vi "RT Main.vi"() -> ()   [LabVIEW 2025]
doc: "This template is for the Queued Message Handler design pattern.\n\nThe Event Handling Loop generates messages based on user interface actions.\n\nThe Message Handling Loop processes messages generated by the Event Handling Loop, or by other messages. The messages are string values, so new messages can be added easily to the Message Cases case structure in the Message Handling Loop. Each message cluster can also provide an optional value for Message Data, which is a variant that can be converted to whatever message-specific data is required."
uses:
  support/Message Queue/Message Queue.lvlib
  controls/Raw Values.ctl
  controls/Control Configuration.ctl
  controls/Control State.ctl
  Globals/Global - Configuration Options.vi
  Globals/Global - RT Stream Connections.vi
  controls/Functional Global Operation.ctl
  C:/40T/controls/Control State.ctl
  <vilib>/nisyscfg/nisyscfg.lvlib
  C:/40T/controls/ProfiBusData.ctl
  controls/ProfiBusData.ctl
panel:
  out "cluster":T1
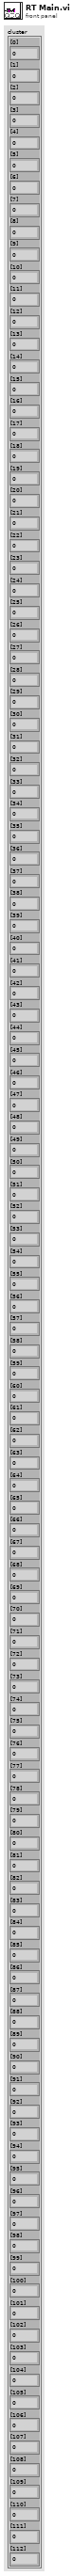
[diagram p1: front panel]
types:
  T1 = typedef "ProfiBusData.ctl" = cluster{"[0]":dbl, "[1]":dbl, "[2]":dbl, "[3]":dbl, "[4]":dbl, "[5]":dbl, "[6]":dbl, "[7]":dbl, "[8]":dbl, "[9]":dbl, "[10]":dbl, "[11]":dbl, "[12]":dbl, "[13]":dbl, "[14]":dbl, "[15]":dbl, "[16]":dbl, "[17]":dbl, "[18]":dbl, "[19]":dbl, "[20]":dbl, "[21]":dbl, "[22]":dbl, "[23]":dbl, "[24]":dbl, "[25]":dbl, "[26]":dbl, "[27]":dbl, "[28]":dbl, "[29]":dbl, "[30]":dbl, "[31]":dbl, "[32]":dbl, "[33]":dbl, "[34]":dbl, "[35]":dbl, "[36]":dbl, "[37]":dbl, "[38]":dbl, "[39]":dbl, "[40]":dbl, "[41]":dbl, "[42]":dbl, "[43]":dbl, "[44]":dbl, "[45]":dbl, "[46]":dbl, "[47]":dbl, "[48]":dbl, "[49]":dbl, "[50]":dbl, "[51]":dbl, "[52]":dbl, "[53]":dbl, "[54]":dbl, "[55]":dbl, "[56]":dbl, "[57]":dbl, "[58]":dbl, "[59]":dbl, "[60]":dbl, "[61]":dbl, "[62]":dbl, "[63]":dbl, "[64]":dbl, "[65]":dbl, "[66]":dbl, "[67]":dbl, "[68]":dbl, "[69]":dbl, "[70]":dbl, "[71]":dbl, "[72]":dbl, "[73]":dbl, "[74]":dbl, "[75]":dbl, "[76]":dbl, "[77]":dbl, "[78]":dbl, "[79]":dbl, "[80]":dbl, "[81]":dbl, "[82]":dbl, "[83]":dbl, "[84]":dbl, "[85]":dbl, "[86]":dbl, "[87]":dbl, "[88]":dbl, "[89]":dbl, "[90]":dbl, "[91]":dbl, "[92]":dbl, "[93]":dbl, "[94]":dbl, "[95]":dbl, "[96]":dbl, "[97]":dbl, "[98]":dbl, "[99]":dbl, "[100]":dbl, "[101]":dbl, "[102]":dbl, "[103]":dbl, "[104]":dbl, "[105]":dbl, "[106]":dbl, "[107]":dbl, "[108]":dbl, "[109]":dbl, "[110]":dbl, "[111]":dbl, "[112]":dbl}
  T2 = typedef "Functional Global Operation.ctl" = enum16{"Initialize", "Read", "Write"}
  T3 = typedef "Control State.ctl" = enum16{"Safe State", "Control (PID)"}
  T4 = typedef "Raw Values.ctl" = cluster{"Channel 0":dbl, "Channel 1":dbl, "Channel 2":dbl, "Channel 3":dbl}
  T5 = typedef "Control Configuration.ctl" = cluster{"PID Gains":cluster{"proportional gain (Kc)":dbl, "integral gain (Kc*Ts/Ti)":dbl, "derivative gain (Kc*Td/Ts)":dbl}, "Output Range":cluster{"output high":dbl, "output low":dbl}}
  T6 = typedef "All Control Configuration Values.ctl" = cluster{"Control State":T3, "Setpoints":T4, "Control Configurations":T5[], "Temperature Thresholds":dbl[]}
  T7 = cluster{"[0]":dbl, "[1]":dbl, "[2]":dbl, "[3]":dbl, "[4]":dbl, "[5]":dbl, "[6]":dbl, "[7]":dbl, "[8]":dbl, "[9]":dbl, "[10]":dbl, "[11]":dbl, "[12]":dbl, "[13]":dbl, "[14]":dbl, "[15]":dbl, "[16]":dbl, "[17]":dbl, "[18]":dbl, "[19]":dbl, "[20]":dbl, "[21]":dbl, "[22]":dbl, "[23]":dbl, "[24]":dbl, "[25]":dbl, "[26]":dbl, "[27]":dbl, "[28]":dbl, "[29]":dbl, "[30]":dbl, "[31]":dbl, "[32]":dbl, "[33]":dbl, "[34]":dbl, "[35]":dbl, "[36]":dbl, "[37]":dbl, "[38]":dbl, "[39]":dbl, "[40]":dbl, "[41]":dbl, "[42]":dbl, "[43]":dbl, "[44]":dbl, "[45]":dbl, "[46]":dbl, "[47]":dbl, "[48]":dbl, "[49]":dbl, "[50]":dbl, "[51]":dbl, "[52]":dbl, "[53]":dbl, "[54]":dbl, "[55]":dbl, "[56]":dbl, "[57]":dbl, "[58]":dbl, "[59]":dbl, "[60]":dbl, "[61]":dbl, "[62]":dbl, "[63]":dbl, "[64]":dbl, "[65]":dbl, "[66]":dbl, "[67]":dbl, "[68]":dbl, "[69]":dbl, "[70]":dbl, "[71]":dbl, "[72]":dbl, "[73]":dbl, "[74]":dbl, "[75]":dbl, "[76]":dbl, "[77]":dbl, "[78]":dbl, "[79]":dbl, "[80]":dbl, "[81]":dbl, "[82]":dbl, "[83]":dbl, "[84]":dbl, "[85]":dbl, "[86]":dbl, "[87]":dbl, "[88]":dbl, "[89]":dbl, "[90]":dbl, "[91]":dbl, "[92]":dbl, "[93]":dbl, "[94]":dbl, "[95]":dbl, "[96]":dbl, "[97]":dbl, "[98]":dbl, "[99]":dbl, "[100]":dbl, "[101]":dbl, "[102]":dbl, "[103]":dbl, "[104]":dbl, "[105]":dbl, "[106]":dbl, "[107]":dbl, "[108]":dbl, "[109]":dbl, "[110]":dbl, "[111]":dbl, "[112]":dbl}
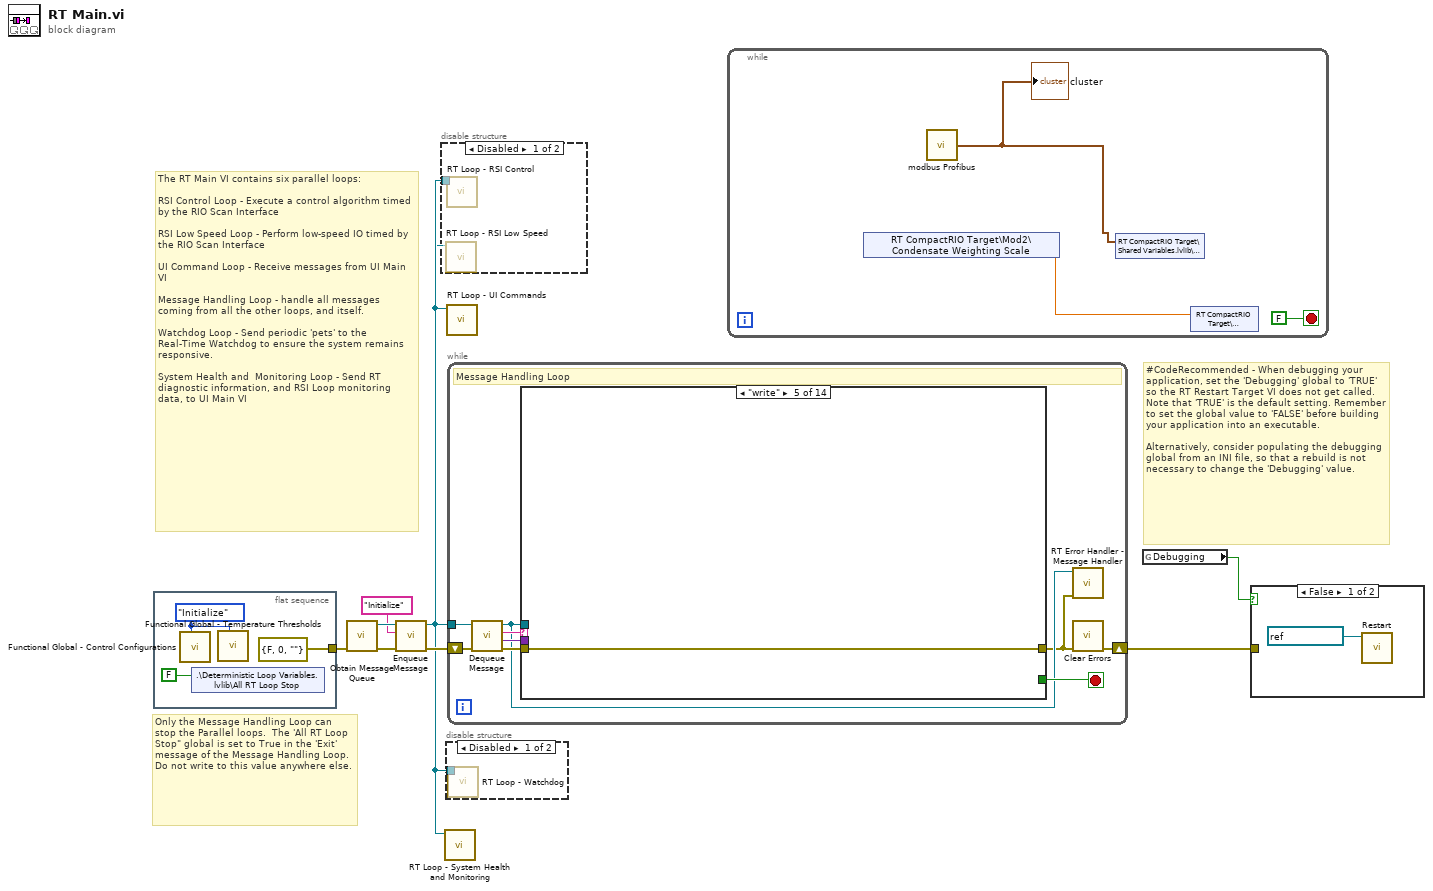
[diagram p0: block diagram]
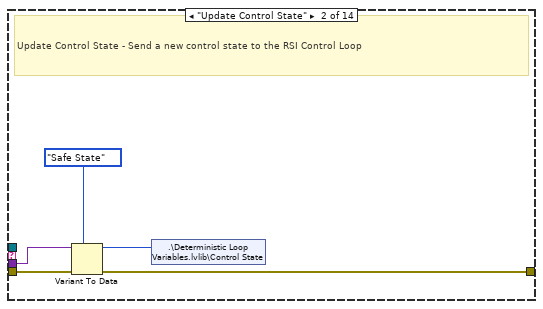
[diagram p6: hidden frame]
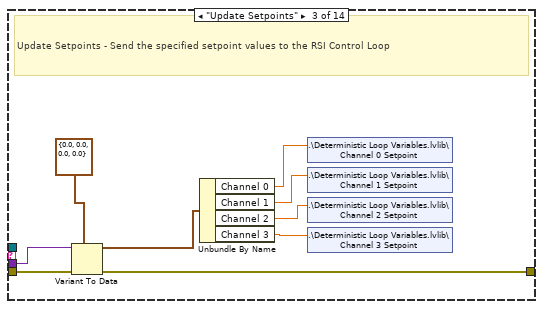
[diagram p7: hidden frame]
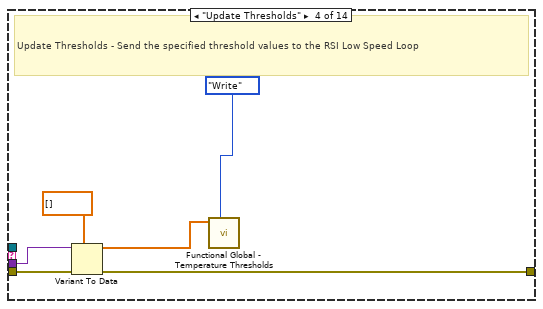
[diagram p8: hidden frame]
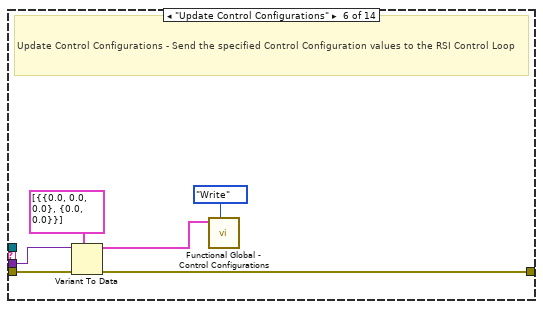
[diagram p9: hidden frame]
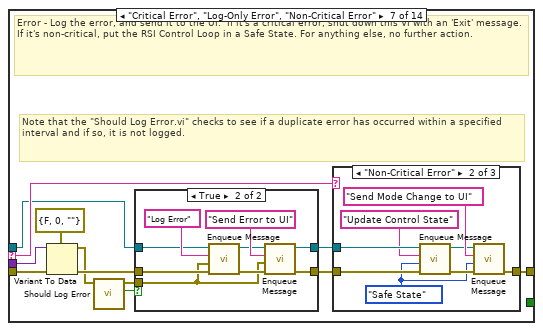
[diagram p10: hidden frame]
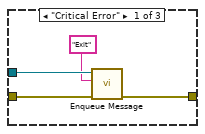
[diagram p12: hidden frame]
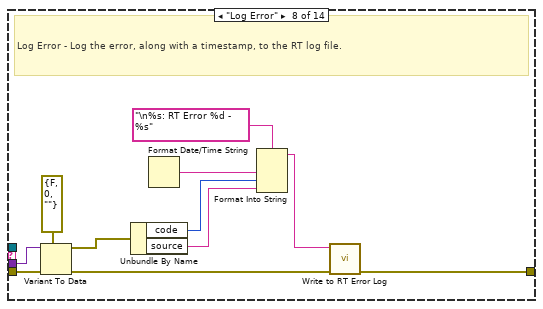
[diagram p14: hidden frame]
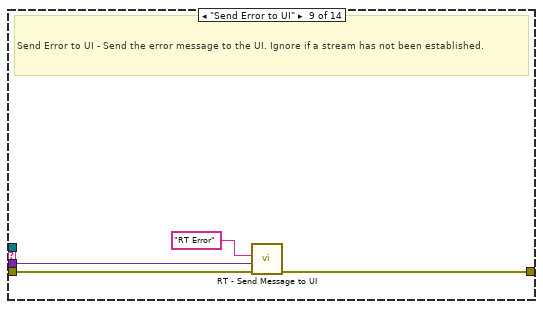
[diagram p15: hidden frame]
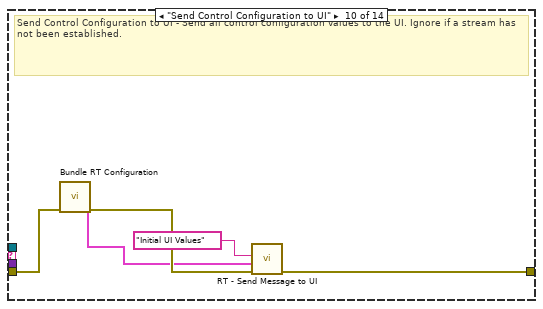
[diagram p16: hidden frame]
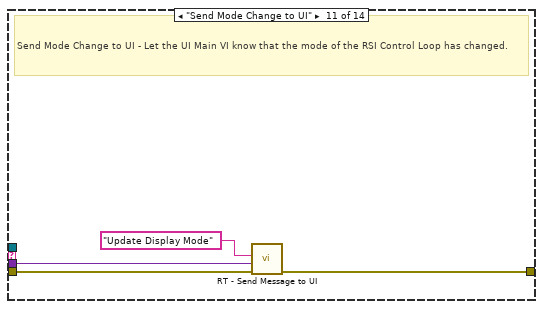
[diagram p17: hidden frame]
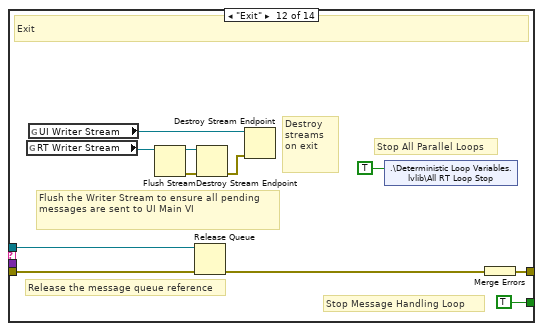
[diagram p18: hidden frame]
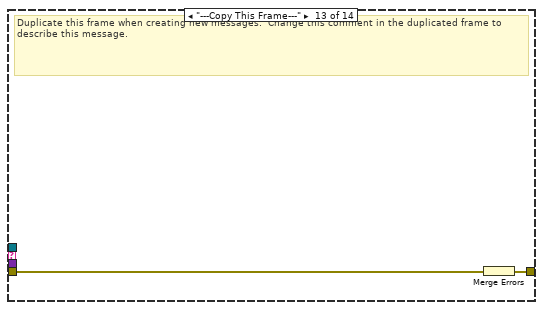
[diagram p19: hidden frame]
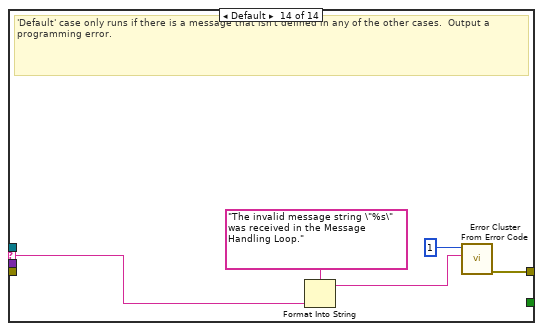
[diagram p20: hidden frame]
diagram:
  # "#CodeRecommended - When debugging your application, set the 'Debugging' global to 'TRUE' so the RT Restart Target VI does not get called.  Note that 'TRUE' is the default setting. Remember to set the global value to 'FALSE' before building your application into an executable.\n\nAlternatively, consider populating the debugging global from an INI file, so that a rebuild is not necessary to change the 'Debugging' value."
  # "The RT Main VI contains six parallel loops:\n\nRSI Control Loop - Execute a control algorithm timed by the RIO Scan Interface\n\nRSI Low Speed Loop - Perform low-speed IO timed by the RIO Scan Interface\n\nUI Command Loop - Receive messages from UI Main VI\n\nMessage Handling Loop - handle all messages coming from all the other loops, and itself.\n\nWatchdog Loop - Send periodic 'pets' to the Real-Time Watchdog to ensure the system remains responsive.\n\nSystem Health and  Monitoring Loop - Send RT diagnostic information, and RSI Loop monitoring data, to UI Main VI"
  # "Only the Message Handling Loop can stop the Parallel loops.  The 'All RT Loop Stop\" global is set to True in the 'Exit' message of the Message Handling Loop.  Do not write to this value anywhere else."
  n1 = flat-sequence {
    tunnel: [errorcluster {"status"=FALSE, "code"=0, "source"=""} ("error constant")] -> w4
    frame #0 {
      w10 = Functional_Global_Operation."Initialize" ("Functional Global Operation (Read)")
      n2 = call "Functional Global - Control Configurations.vi"("Functional Global Operation (Read)"=w10) -> ()  [unwired: 10 in, 1 out]
      n3 = shared-variable ".\\Deterministic Loop Variables.lvlib\\All RT Loop Stop"(FALSE) -> ()  [unwired: 1 in, 1 out]
      n4 = call "Functional Global - Temperature Thresholds.vi"("Functional Global Operation (Read)"=w10) -> ()  [unwired: 10 in, 1 out]
    }
  }
  n5 = call "Obtain Message Queue.vi"("error in (no error)"=w4) -> ("error out"=w1:errorcluster, "Message Queue"=w8:refnum<queue>)  [unwired: 9 in]
  n6 = call "Enqueue Message.vi"("error in (no error)"=w1, "Message"="Initialize", "Message Queue"=w8) -> ("error out"=w6:errorcluster, "dup Message Queue"=w2:refnum<queue>)  [unwired: 7 in]
  n7 = disable-structure shown="Disabled" {
    disable-tunnel: w2 -> [w12 _]
    frame Disabled {
      n8 = call "RT Loop - RSI Low Speed.vi"("Message Queue"=w12) -> ()  [unwired: 11 in]
      n9 = call "RT Loop - RSI Control.vi"("Message Queue"=w12) -> ()  [unwired: 11 in]
    }
    frame Enabled {
    }
  }
  n10 = call "RT Loop - System Health and Monitoring.vi"("Message Queue"=w2) -> ()  [unwired: 11 in]
  n11 = call "RT Loop - UI Commands.vi"("Message Queue"=w2) -> ()  [unwired: 11 in]
  n12 = disable-structure shown="Disabled" {
    disable-tunnel: w2 -> [w13 _]
    frame Disabled {
      n13 = call "RT Loop - Watchdog.vi"("Message Queue"=w13) -> ()  [unwired: 11 in]
    }
    frame Enabled {
    }
  }
  n14 = while {
    tunnel: w2 -> [w17]
    shift-right: [w15] -> w3
    shift-left: w6 -> [w21]
    stop <- w22 stop-if-true
    # "Message Handling Loop"
    n15 = call "Dequeue Message.vi"("error in (no error)"=w21, "Message Queue"=w17) -> ("error out"=w20:errorcluster, "Message Data"=w18:variant, "Message"=w19:string, "dup Message Queue"=w16:refnum<queue>)  [unwired: 6 in]
    n16 = case "Message Cases" shown="\"write\"" w19 {
      selector: w19 -> [_ _ _ _ _ _ w60 _ _ _ _ _ _ w127]
      tunnel: w16 -> [_ _ _ _ _ _ w54 _ _ _ _ w121 _ _]
      tunnel: w20 -> [w23 w28 w37 w43 w44 w50 w58 w97 w101 w106 w110 w117 w123 _]
      tunnel: [w23 w25 w29 w41 w44 w47 w59 w88 w98 w102 w109 w118 w122 w125] -> w14
      tunnel: [_ _ _ _ _ _ _ _ _ _ _ TRUE _ _] -> w22
      tunnel: w18 -> [_ w27 w36 w42 _ w49 w57 w96 w100 _ w108 _ _ _]
      frame "Initialize" {
        # "Initialize - Currently a no-op for the RT Main VI"
      }
      frame "Update Control State" {
        # "Update Control State - Send a new control state to the RSI Control Loop"
        n17 = Variant To Data(error in=w28, type=Control_State."Safe State" ("FPGA State"), Variant=w27) -> (data=w24:T3, error out=w25:errorcluster)
        n18 = shared-variable ".\\Deterministic Loop Variables.lvlib\\Control State"(w24) -> ()  [unwired: 1 in, 1 out]
      }
      frame "Update Setpoints" {
        # "Update Setpoints - Send the specified setpoint values to the RSI Control Loop"
        n19 = Variant To Data(error in=w37, type=T4 {"Channel 0"=0.0, "Channel 1"=0.0, "Channel 2"=0.0, "Channel 3"=0.0} ("Raw Values"), Variant=w36) -> (data=w34:T4, error out=w29:errorcluster)
        n20 = Unbundle By Name(w34) -> ("Channel 0"=w30:dbl, "Channel 1"=w31:dbl, "Channel 2"=w32:dbl, "Channel 3"=w33:dbl)
        n21 = shared-variable ".\\Deterministic Loop Variables.lvlib\\Channel 0 Setpoint"(w30) -> ()  [unwired: 1 in, 1 out]
        n22 = shared-variable ".\\Deterministic Loop Variables.lvlib\\Channel 1 Setpoint"(w31) -> ()  [unwired: 1 in, 1 out]
        n23 = shared-variable ".\\Deterministic Loop Variables.lvlib\\Channel 2 Setpoint"(w32) -> ()  [unwired: 1 in, 1 out]
        n24 = shared-variable ".\\Deterministic Loop Variables.lvlib\\Channel 3 Setpoint"(w33) -> ()  [unwired: 1 in, 1 out]
      }
      frame "Update Thresholds" {
        # "Update Thresholds - Send the specified threshold values to the RSI Low Speed Loop"
        n25 = Variant To Data(error in=w43, type=dbl[] [], Variant=w42) -> (data=w38:dbl[], error out=w41:errorcluster)
        n26 = call "Functional Global - Temperature Thresholds.vi"("Functional Global Operation (Read)"=Functional_Global_Operation."Write", "Temperature Thresholds in"=w38) -> ()  [unwired: 9 in, 1 out]
      }
      frame "write" {
      }
      frame "Update Control Configurations" {
        # "Update Control Configurations - Send the specified Control Configuration values to the RSI Control Loop"
        n27 = Variant To Data(error in=w50, type=T5[] [{"PID Gains"={"proportional gain (Kc)"=0.0, "integral gain (Kc*Ts/Ti)"=0.0, "derivative gain (Kc*Td/Ts)"=0.0}, "Output Range"={"output high"=0.0, "output low"=0.0}}], Variant=w49) -> (data=w46:T5[], error out=w47:errorcluster)
        n28 = call "Functional Global - Control Configurations.vi"("Functional Global Operation (Read)"=Functional_Global_Operation."Write", "Control Configurations in"=w46) -> ()  [unwired: 9 in, 1 out]
      }
      frame "Critical Error", "Log-Only Error", "Non-Critical Error" {
        # "Note that the \"Should Log Error.vi\" checks to see if a duplicate error has occurred within a specified interval and if so, it is not logged."
        # "Error - Log the error, and send it to the UI.  If it's a critical error, shut down this VI with an 'Exit' message. If it's non-critical, put the RSI Control Loop in a Safe State. For anything else, no further action."
        n29 = Variant To Data(error in=w58, type=errorcluster {"status"=FALSE, "code"=0, "source"=""} ("error out"), Variant=w57) -> (data=w52:errorcluster, error out=w55:errorcluster)
        n30 = call "Should Log Error.vi"("error to report"=w52) -> ("Should Log Error?"=w53:bool, "dup error to report"=w51:errorcluster)  [unwired: 9 in]
        n31 = case shown="True" w53 {
          tunnel: [w64 w71] -> w62
          tunnel: [w63 w70] -> w61
          tunnel: w54 -> [w63 w69]
          tunnel: w55 -> [w64 w66]
          tunnel: w51 -> [_ w65]
          frame False {
          }
          frame True {
            n32 = call "Enqueue Message.vi"("error in (no error)"=w66, "Message Data"=w65, "Message"="Log Error", "Message Queue"=w69) -> ("error out"=w67:errorcluster, "dup Message Queue"=w68:refnum<queue>)  [unwired: 6 in]
            n33 = call "Enqueue Message.vi"("error in (no error)"=w67, "Message Data"=w65, "Message"="Send Error to UI", "Message Queue"=w68) -> ("error out"=w71:errorcluster, "dup Message Queue"=w70:refnum<queue>)  [unwired: 6 in]
          }
        }
        n34 = case shown="\"Non-Critical Error\"" w60 {
          tunnel: w62 -> [w77 w85 w86]
          tunnel: w61 -> [w75 w84 _]
          tunnel: [w76 w81 w86] -> w59
          frame "Critical Error" {
            n35 = call "Enqueue Message.vi"("error in (no error)"=w77, "Message"="Exit", "Message Queue"=w75) -> ("error out"=w76:errorcluster)  [unwired: 7 in, 1 out]
          }
          frame "Non-Critical Error" {
            w78 = Control_State."Safe State" ("FPGA State")
            n36 = call "Enqueue Message.vi"("error in (no error)"=w85, "Message Data"=w78, "Message"="Update Control State", "Message Queue"=w84) -> ("error out"=w82:errorcluster, "dup Message Queue"=w79:refnum<queue>)  [unwired: 6 in]
            n37 = call "Enqueue Message.vi"("error in (no error)"=w82, "Message Data"=w78, "Message"="Send Mode Change to UI", "Message Queue"=w79) -> ("error out"=w81:errorcluster)  [unwired: 6 in, 1 out]
          }
          frame Default {
          }
        }
      }
      frame "Log Error" {
        # "Log Error - Log the error, along with a timestamp, to the RT log file."
        n38 = Variant To Data(error in=w97, type=errorcluster {"status"=FALSE, "code"=0, "source"=""} ("error constant"), Variant=w96) -> (data=w91:errorcluster, error out=w94:errorcluster)
        n39 = Unbundle By Name(w91) -> ("code"=w90:i32, "source"=w89:string)
        n40 = Format Date/Time String() -> (date/time string=w92:string)  [unwired: 3 in]
        n41 = Format Into String(format string="\n%s: RT Error %d - %s", w92, w90, w89) -> (resulting string=w87:string)  [unwired: 2 in, 1 out]
        n42 = call "Write to RT Error Log.vi"("error in (no error)"=w94, "Log Entry"=w87) -> ("error out"=w88:errorcluster)  [unwired: 9 in]
      }
      frame "Send Error to UI" {
        # "Send Error to UI - Send the error message to the UI. Ignore if a stream has not been established."
        n43 = call "RT - Send Message to UI.vi"("error in (no error)"=w101, "Message Data"=w100, "Message"="RT Error") -> ("error out"=w98:errorcluster)  [unwired: 8 in]
      }
      frame "Send Control Configuration to UI" {
        # "Send Control Configuration to UI - Send all control configuration values to the UI. Ignore if a stream has not been established."
        n44 = call "Bundle RT Configuration.vi"("error in (no error)"=w106) -> ("error out"=w105:errorcluster, "All Control Configuration Values"=w104:T6)  [unwired: 9 in]
        n45 = call "RT - Send Message to UI.vi"("error in (no error)"=w105, "Message Data"=w104, "Message"="Initial UI Values") -> ("error out"=w102:errorcluster)  [unwired: 8 in]
      }
      frame "Send Mode Change to UI" {
        # "Send Mode Change to UI - Let the UI Main VI know that the mode of the RSI Control Loop has changed."
        n46 = call "RT - Send Message to UI.vi"("error in (no error)"=w110, "Message Data"=w108, "Message"="Update Display Mode") -> ("error out"=w109:errorcluster)  [unwired: 8 in]
      }
      frame "Exit" {
        # "Flush the Writer Stream to ensure all pending messages are sent to UI Main VI"
        # "Destroy streams on exit"
        # "Stop Message Handling Loop"
        # "Stop All Parallel Loops"
        # "Release the message queue reference"
        # "Exit"
        n47 = global read "Global - RT Stream Connections.vi" "RT Writer Stream"() -> (w116:refnum<k21>)
        n48 = global read "Global - RT Stream Connections.vi" "UI Writer Stream"() -> (w115:refnum<k21>)
        n49 = Flush Stream(11:w116) -> (0:w111:errorcluster, 3:w112:refnum<k21>)  [unwired: 3 in, 1 out]
        n50 = Release Queue(queue=w121, error in (no error)=w117) -> (error out=w119:errorcluster)  [unwired: 1 in, 2 out]
        n51 = Destroy Stream Endpoint(8:w111, 11:w112) -> (0:w114:errorcluster)
        n52 = Destroy Stream Endpoint(8:w114, 11:w115) -> ()  [unwired: 1 out]
        n53 = shared-variable ".\\Deterministic Loop Variables.lvlib\\All RT Loop Stop"(TRUE ("Stop Monitoring Loops")) -> ()  [unwired: 1 in, 1 out]
        n54 = Merge Errors(w119) -> (w118:errorcluster)
      }
      frame "---Copy This Frame---" {
        # "Duplicate this frame when creating new messages.  Change this comment in the duplicated frame to describe this message."
        n55 = Merge Errors(w123) -> (w122:errorcluster)
      }
      frame Default {
        # "'Default' case only runs if there is a message that isn't defined in any of the other cases.  Output a programming error."
        n56 = Format Into String(format string="The invalid message string \"%s\" was received in the Message Handling Loop." ("Unknown Message Error Text"), w127) -> (resulting string=w124:string)  [unwired: 2 in, 1 out]
        n57 = call <vilib>:"Error Cluster From Error Code.vi"("error message (\"\")"=w124, "error code (0)"=1) -> ("error out"=w125:errorcluster)  [unwired: 7 in]
      }
    }
    n58 = call "RT Error Handler - Message Handler.vi"("error in (no error)"=w14, "Message Queue"=w16) -> ()  [unwired: 9 in, 1 out]
    n59 = call <vilib>:"Clear Errors.vi"("error in (no error)"=w14) -> ("error out"=w15:errorcluster)  [unwired: 5 in, 1 out]
  }
  n60 = while {
    stop <- FALSE stop-if-true
    n61 = shared-variable "RT CompactRIO Target\\Mod2\\Condensate Weighting Scale"() -> (w130:dbl)  [unwired: 1 in, 1 out]
    n62 = call "modbus Profibus.vi"() -> ("cluster"=w129:T7)  [unwired: 12 in, 3 out]
    "cluster" <- w129
    n63 = shared-variable "RT CompactRIO Target\\Shared Variables.lvlib\\Profibus"(w129) -> ()  [unwired: 1 in, 1 out]
    n64 = shared-variable "RT CompactRIO Target\\Deterministic Loop Variables.lvlib\\AO1"(w130) -> ()  [unwired: 1 in, 1 out]
  }
  n65 = global read "Global - Configuration Options.vi" "Debugging"() -> (w5:bool)
  n66 = case shown="False" w5 {
    tunnel: w3 -> [_ _]
    frame False {
      n67 = call <vilib>:"Restart.vi"("Session in"=refnum<k21> "localhost" ("session in")) -> ()  [unwired: 8 in, 3 out]
    }
    frame True {
    }
  }
